vi "Gain Add or Remove.vi"(8 "error in (no error)":errorcluster, 9 "Name Prefix":string, 10 "Size":i32, 11 "Channel Gain":T1) -> (0 "error out":errorcluster, 3 "Channel Gain out":T1)   [LabVIEW 2019, in "Instrument.Lockin.lvlib" / "Instrument.DAQ.lvclass"]
uses:
  Instrument.DAQ.lvclass
  Typedefs/Channel.Gain--Cluster--Array.ctl
  Typedefs/Channel.Gain--Cluster.ctl
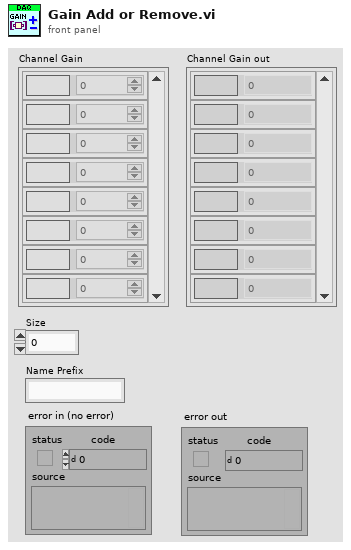
[diagram p1: front panel]
types:
  T1 = typedef "Instrument.Lockin.lvlib/Instrument.DAQ.lvclass/Channel.Gain--Cluster--Array.ctl" = T2[]
  T2 = typedef "Instrument.Lockin.lvlib/Instrument.DAQ.lvclass/Channel.Gain--Cluster.ctl" = cluster{"Channel":string, "Gain":dbl}
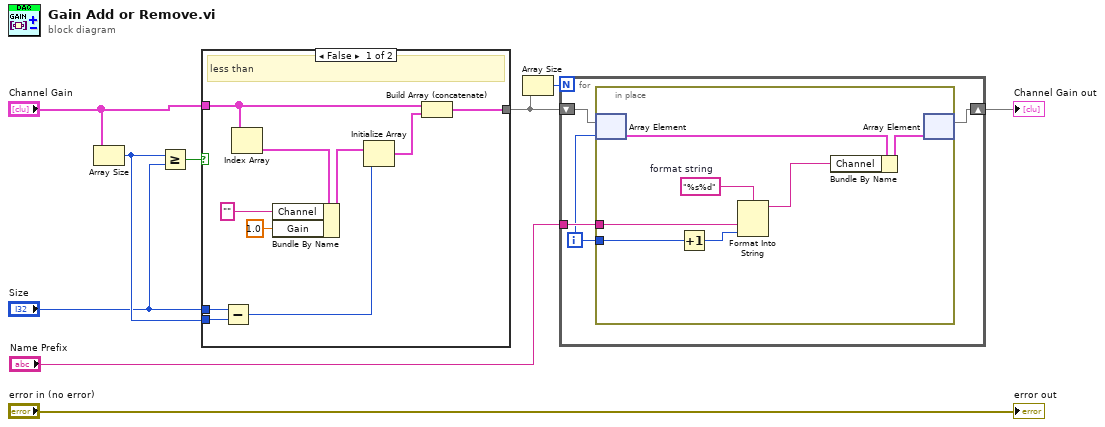
[diagram p0: block diagram]
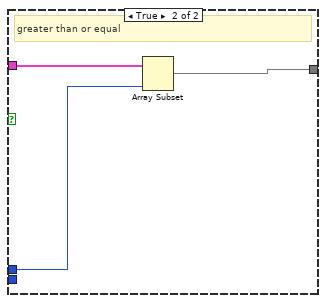
[diagram p2: hidden frame]
diagram:
  n1 = Array Size(array="Channel Gain") -> (size(s)=w9:i32)
  n2 = Greater Or Equal?(x=w9, y="Size") -> (x >= y?=w8:bool)
  n3 = case shown="False" w8 {
    tunnel: "Channel Gain" -> [w13 w22]
    tunnel: "Size" -> [w17 w21]
    tunnel: [w18 w20] -> w2
    tunnel: w9 -> [w16 _]
    frame False {
      # "less than"
      n4 = Subtract(x=w17, y=w16) -> (x-y=w15:i32)
      n5 = Index Array(array=w13) -> (element=w12:T2)  [unwired: 1 in]
      n6 = Bundle By Name(cluster=w12, "Channel"="", "Gain"=1.0) -> (w14:T2)
      n7 = Initialize Array(w14, w15) -> (w19:T2[])
      n8 = Build Array (concatenate)(w13, w19) -> (w18:T1)
    }
    frame True {
      # "greater than or equal"
      n9 = Array Subset(array=w22, length=w21) -> (w20:T1)  [unwired: 1 in]
    }
  }
  n10 = Array Size(array=w2) -> (size(s)=w3:i32)
  n11 = for {
    N: w3 -> [_]
    tunnel: "Name Prefix" -> [w26]
    shift-right: [w25] -> w6
    shift-left: w2 -> [w23]
    i -> [w24]
    n12 = in-place {
      in-place-border: w24 -> [w33]
      in-place-border: w26 -> [w30]
      w32 = "%s%d"  # format string
      n13 = in-place-array #1(w23, w24) -> (w29:T2)
      n14 = Increment(x=w33) -> (x+1=w31:i32)
      n15 = Format Into String(format string=w32, w30, w31) -> (resulting string=w27:string)  [unwired: 2 in, 1 out]
      n16 = Bundle By Name(cluster=w29, "Channel"=w27) -> (w28:T2)
      n17 = in-place-array #1(w28) -> (w25:T1)  [unwired: 1 out]
    }
  }
  "Channel Gain out" <- w6
  "error out" <- "error in (no error)"
